vi "Configure Module.vi"(8 "error in (no error)":errorcluster, 10 "IOV ref in":variant, 11 "Module Template in":refnum<class "9401.lvclass">) -> (0 "error out":errorcluster, 2 "IOV ref out":variant, 3 "Module Template out":refnum<class "9401.lvclass">)   [LabVIEW 2020, in "Modules.lvlib" / "9401.lvclass"]
uses:
  9401.lvclass
  <resource>/objmgr/cRIO.rc
  SD Module/SD Module.lvclass
  C:/Users/nitest/Desktop/Git 2020/niveristand-scan-engine-module-libraries/Source/SD Module/SD Module.lvclass
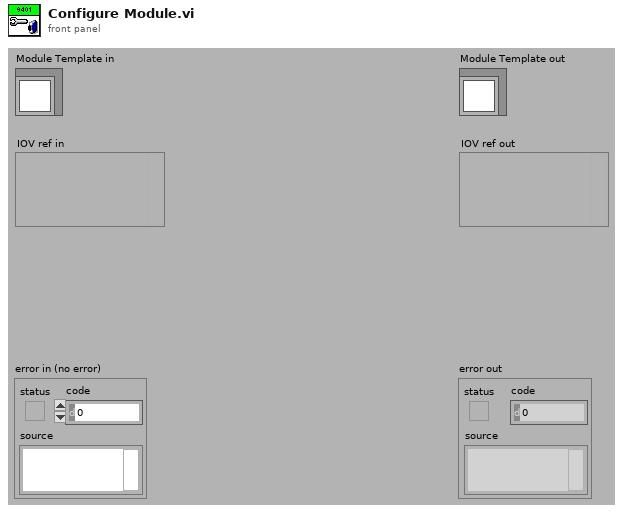
[diagram p1: front panel]
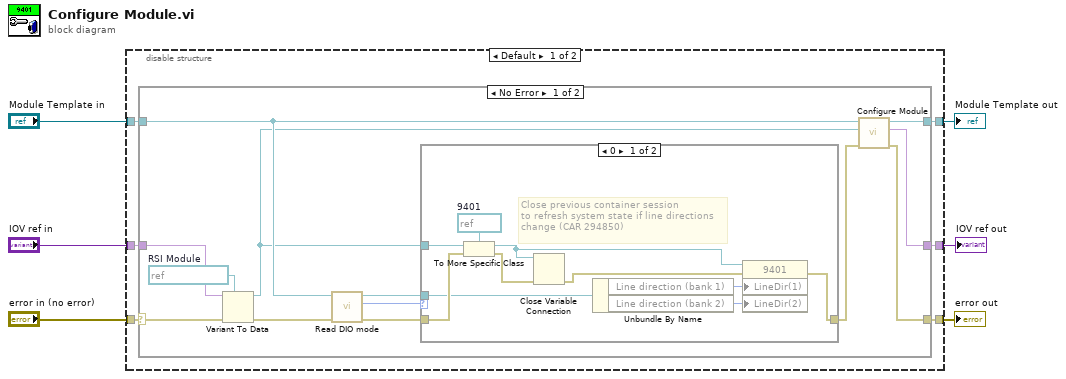
[diagram p0: block diagram]
diagram:
  n1 = disable-structure shown="Default" {
    disable-tunnel: "error in (no error)" -> [w12 w42]
    disable-tunnel: [w11 w42] -> w5
    disable-tunnel: "Module Template in" -> [w10 w40]
    disable-tunnel: [w9 w40] -> w3
    disable-tunnel: "IOV ref in" -> [w8 w41]
    disable-tunnel: [w7 w41] -> w1
    frame condition #0 {
      n2 = case shown="No Error" w12 {
        selector: w12 -> [w16 w39]
        tunnel: [w21 w39] -> w11
        tunnel: [w18 w38] -> w9
        tunnel: w10 -> [w20 w38]
        tunnel: w8 -> [w17 w37]
        tunnel: [w19 w37] -> w7
        frame No Error {
          w14 = refnum<k21> refnum  # RSI Module
          n3 = Variant To Data(error in=w16, type=w14, Variant=w17) -> (data=w13:refnum<k21>, error out=w15:errorcluster)
          n4 = call "Read DIO mode.vi"("error in (no error)"=w15, "SD Module in"=w20) -> ("error out"=w23:errorcluster, "DIO mode"=w24:u32, "SD Module out"=w25:refnum<class "9401.lvclass">)  [unwired: 7 in]
          n5 = case shown="0" w24 {
            tunnel: [w26 w36] -> w22
            tunnel: w13 -> [w34 _]
            tunnel: w25 -> [w27 _]
            tunnel: w23 -> [w28 w36]
            frame 0 {
              w35 = refnum<k21> refnum  # 9401
              # "Close previous container session\nto refresh system state if line directions\nchange (CAR 294850)"
              n6 = To More Specific Class(target class=w35, reference=w34, error in=w28) -> (specific class reference=w29:refnum<k21>, error out=w31:errorcluster)
              n7 = Close Variable Connection(8:w31, 11:w29) -> (0:w30:errorcluster)
              n8 = Unbundle By Name(w27) -> ("Line direction (bank 1)"=w33:u32, "Line direction (bank 2)"=w32:u32)
              n9 = property class="9401"(reference=w29, error in=w30, "LineDir(1)"=w33, "LineDir(2)"=w32) -> (error out=w26:errorcluster)  [unwired: 1 out]
            }
            frame Default {
            }
          }
          n10 = call-parent "Configure Module.vi"("error in (no error)"=w22, "IOV ref in"=w13, "Module Template in"=w20) -> ("error out"=w21:errorcluster, "IOV ref out"=w19:variant, "Module Template out"=w18:refnum<class "9401.lvclass">)  [unwired: 6 in]
        }
        frame Error {
        }
      }
    }
    frame condition #1 (active) {
    }
  }
  "error out" <- w5
  "Module Template out" <- w3
  "IOV ref out" <- w1
